vi "RemoteVI Fixture Key Line.vi"(0 "CtlRef":refnum<vi>, 1 "Char":i16, 2 "VKey":string, 3 "PlatMods":T1, 5 "error in":errorcluster) -> (14 "line":string, 19 "error out":errorcluster)   [LabVIEW 2020]
doc: "Event-log helper of RemoteVI Fixture.vi. Builds one key line of the log: keydown TAB label TAB key TAB mods LF, where label is read from the event's control reference, key is the typed character when Char is printable (32 to 126) and the VKey name otherwise, and mods the held modifiers as RemoteVI Fixture Mods.vi writes them. Errors of reading the label go to error out."
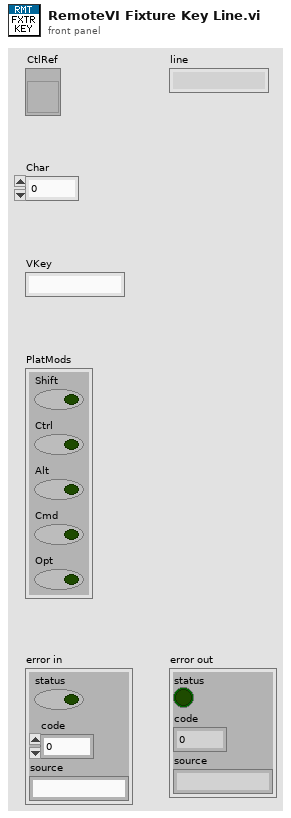
[diagram p1: front panel]
types:
  T1 = cluster{"Shift":bool, "Ctrl":bool, "Alt":bool, "Cmd":bool, "Opt":bool}
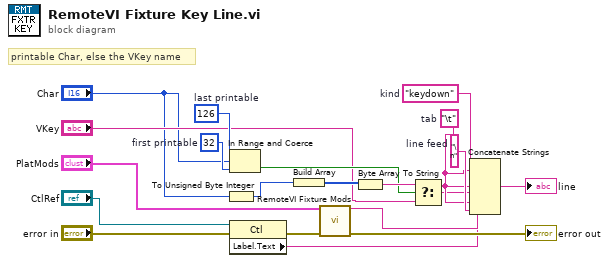
[diagram p0: block diagram]
diagram:
  w19 = "\n"  # line feed
  w18 = "\t"  # tab
  w17 = "keydown"  # kind
  w9 = i16 32  # first printable
  w8 = i16 126  # last printable
  # "printable Char, else the VKey name"
  n1 = To Unsigned Byte Integer(number="Char") -> (unsigned 8bit integer=w11:u8)
  n2 = In Range and Coerce(upper limit=w8, x="Char", lower limit=w9) -> (In Range?=w10:bool)  [unwired: 1 out]
  n3 = property class="Ctl"(reference="CtlRef", error in="error in") -> (error out=w7:errorcluster, "Label.Text"=w6:string)  [unwired: 1 out]
  n4 = Build Array(w11) -> (w12:u8[])
  n5 = call "RemoteVI Fixture Mods.vi"("PlatMods"="PlatMods", "error in"=w7) -> ("mods"=w15:string, "error out"=→"error out":errorcluster)  [unwired: 12 in]
  n6 = Byte Array To String(unsigned byte array=w12) -> (string=w13:string)
  n7 = Select(t=w13, s=w10, f="VKey") -> (s? t:f=w14:string)
  n8 = Concatenate Strings(w17, w18, w6, w18, w14, w18, w15, w19) -> (→"line":string)
